vi "FuncVI2-Call.vi"(4 "Caller CSE RefNum":T1, 5 "InstanceRef":T3, 9 "arg list":T2[](array[typedef]) {"num" format="%.2f"}) -> (0 "error out":bool, 3 "result":T2 {"num" format="%.2f"})   [LabVIEW 2021]
doc: "::: CalcExpress Toolkit :::\nCopyright (c) 2000-2026 Konstantin Shifershteyn. All rights reserved."
uses:
  cetypes.llb/CalcExpress Function Argument Info.ctl
  cetypes.llb/CalcExpress Instance RefNum.ctl
  cse.llb/CSE Instance RefNum.ctl
panel:
  in  "max arg num":i32=1000
  in  "min arg num":i32=1
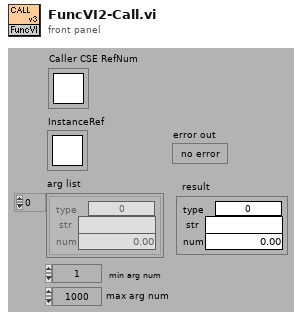
[diagram p1: front panel]
types:
  T1 = typedef "CSE Instance RefNum.ctl" = refnum<k1>
  T2 = typedef "CalcExpress Function Argument Info.ctl" = cluster{"type":u32, "str":string, "num":dbl}
  T3 = typedef "CalcExpress Instance RefNum.ctl" = refnum<k1>
  T4 = enum32{"String", "DBL Number", "identifier", "1D Array of DBL", "2D Array of DBL", "CDB Number", "1D Array of CDB", "2D Array of CDB", "1D Array of String", "2D Array of String", "Unknown data type"}
  T5 = typedef "VarMan Variable Context Handle.ctl" = i32
  T6 = typedef "CSE Callback VI RefNum.ctl" = refnum<vi>
  T7 = cluster{"type: use this constant to specify a predefined type code":enum32{"String", "DBL Number", "identifier", "1D Array of DBL", "2D Array of DBL", "CDB Number", "1D Array of CDB", "2D Array of CDB", "1D Array of String", "2D Array of String", "Unknown data type"}, string, "return value":dbl}
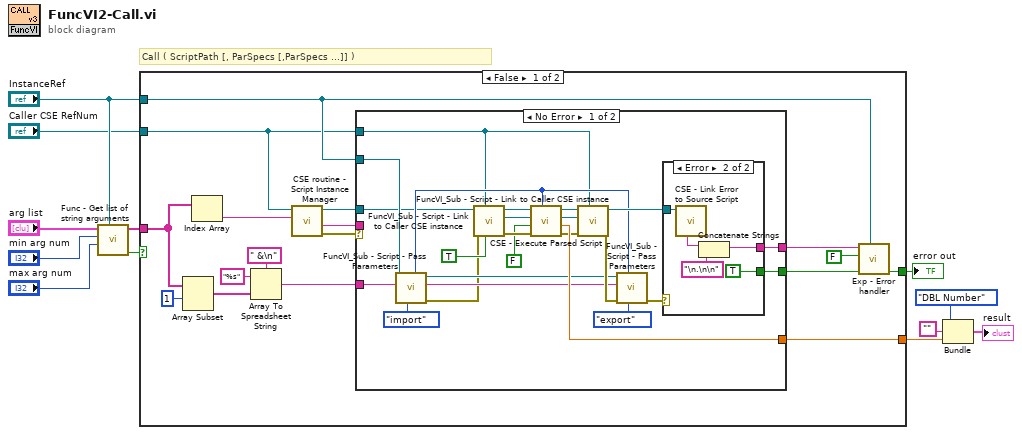
[diagram p0: block diagram]
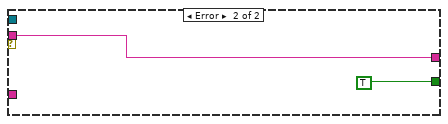
[diagram p3: hidden frame]
diagram:
  # "Call ( ScriptPath [, ParSpecs [,ParSpecs ...]] )"
  n1 = call "Func - Get list of string arguments.vi"("InstanceRef"="InstanceRef", "max arg num"="max arg num", "min arg num"="min arg num", "arg list"="arg list") -> ("error out"=w7:bool, "val list"=w8:string[])  [unwired: 4 in]
  n2 = case shown="False" w7 {
    selector: w7 -> [_ w61]
    tunnel: "InstanceRef" -> [w24 _]
    tunnel: w8 -> [w23 _]
    tunnel: [w28 w61] -> w6
    tunnel: [w29 _] -> w2
    tunnel: "Caller CSE RefNum" -> [w13 _]
    frame False {
      n3 = Array Subset(array=w23, index=1) -> (w19:string[])  [unwired: 1 in]
      n4 = Index Array(array=w23) -> (element=w15:string)  [unwired: 1 in]
      n5 = Array To Spreadsheet String(delimiter (Tab)=" &\n", array=w19, 3:"%s" ("format string")) -> (spreadsheet string=w18:string)
      n6 = call "CSE routine - Script Instance Manager.vi"("Script Name"=w15, "Caller CSE RefNum"=w13) -> ("error out"=w16:errorcluster, "Error message"=w14:string, "new CSE RefNum"=w17:T1)  [unwired: 7 in]
      n7 = case shown="No Error" w16 {
        tunnel: [w53 _] -> w29
        tunnel: [w51 TRUE] -> w27
        tunnel: [w52 w59] -> w26
        tunnel: w13 -> [w33 _]
        tunnel: w18 -> [w36 _]
        tunnel: w24 -> [w35 _]
        tunnel: w17 -> [w32 _]
        tunnel: w14 -> [_ w59]
        frame No Error {
          n8 = call "FuncVI_Sub - Script - Pass Parameters.vi"("action"=enum32{"import", "export"}."import", "parateters specifier"=w36, "CE InstanceRef"=w35) -> ("error out"=w31:errorcluster, "dup parateters specifier"=w37:string, "dup CE InstanceRef"=w39:T3, "Local VC Handle out"=w38:T5)  [unwired: 5 in]
          n9 = call "FuncVI_Sub - Script - Link to Caller CSE instance.vi"("Link(T)/Delink(F)"=TRUE, "Caller CSE RefNum"=w33, "error in"=w31, "CSE RefNum"=w32) -> ("error out"=w45:errorcluster, "Callback VI RefNum out"=w46:T6, "dup CSE RefNum"=w47:T1)  [unwired: 5 in]
          n10 = call "CSE - Execute Parsed Script.vi"("VC Handle"=w38, "error in"=w45, "Close FuncVI Refs (T)"=FALSE, "Callback VI RefNum"=w46, "CSE RefNum"=w47) -> ("error out"=w43:errorcluster, "return value"=w53:dbl, "dup Callback VI RefNum"=w48:T6, "dup CSE RefNum"=w50:T1)  [unwired: 2 in, 1 out]
          n11 = call "FuncVI_Sub - Script - Link to Caller CSE instance.vi"("Caller CSE RefNum"=w33, "error in"=w43, "Callback VI RefNum"=w48, "CSE RefNum"=w50) -> ("error out"=w41:errorcluster, "dup CSE RefNum"=w49:T1)  [unwired: 5 in, 1 out]
          n12 = call "FuncVI_Sub - Script - Pass Parameters.vi"("action"=enum32{"import", "export"}."export", "Local VC Handle"=w38, "error in"=w41, "parateters specifier"=w37, "CE InstanceRef"=w39) -> ("error out"=w42:errorcluster)  [unwired: 3 in, 3 out]
          n13 = case shown="Error" w42 {
            tunnel: w49 -> [_ w58]
            tunnel: [_ TRUE] -> w51
            tunnel: [_ w54] -> w52
            frame No Error {
            }
            frame Error {
              n14 = call "CSE - Link Error to Source Script.vi"("CSE RefNum"=w58) -> ("Error Message"=w56:string)  [unwired: 4 in, 6 out]
              n15 = Concatenate Strings(w56, "\n.\n\n" ("string")) -> (w54:string)
            }
          }
        }
        frame Error {
        }
      }
      n16 = call "Exp - Error handler.vi"("InstanceRef"=w24, "error in"=w27, "add FuncName (T)"=FALSE, "error message in"=w26) -> ("error out"=w28:bool)  [unwired: 5 in, 2 out]
    }
    frame True {
    }
  }
  "error out" <- w6
  n17 = Bundle("type: use this constant to specify a predefined type code"=T4."DBL Number", "", "return value"=w2) -> (→"result":T7)  [unwired: 1 in]
